vi "laser_power_measurement.vi"(1 "stop":bool) -> (0 "Readings":T1(array[cluster]) {"value" format="%#_6p"; "timestamp" format="%#.3f"})   [LabVIEW 2025]
panel:
  out "Device S/Ns":string[](array[string])
  out "Selected device S/N":string
  in  "OphirLMMeasurementLib.ICoLMMeasurement2":refnum<k7>
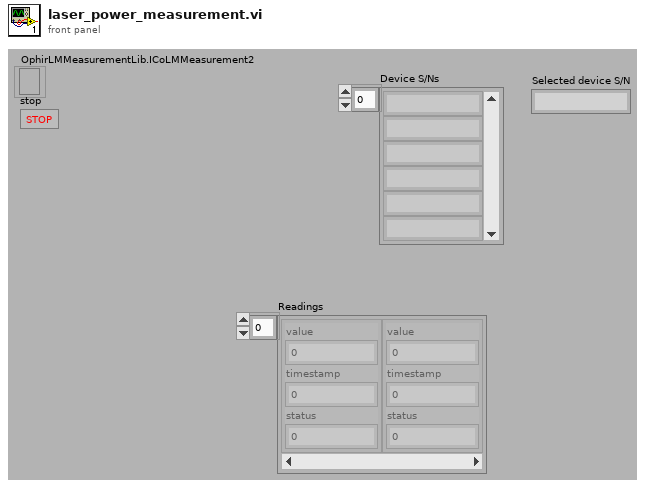
[diagram p1: front panel]
types:
  T1 = cluster{"value":dbl, "timestamp":dbl, "status":i32}[]
  T2 = cluster{"value":dbl, "timestamp":dbl, "status":i32}
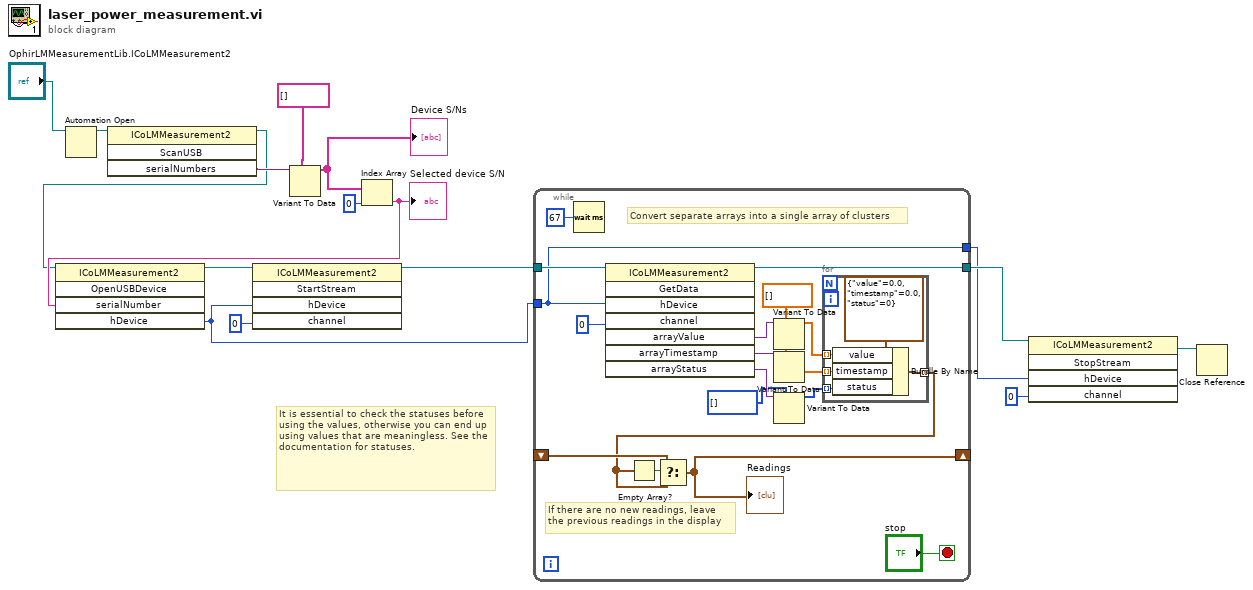
[diagram p0: block diagram]
diagram:
  # "It is essential to check the statuses before using the values, otherwise you can end up using values that are meaningless. See the documentation for statuses."
  n1 = Automation Open(Automation Refnum="OphirLMMeasurementLib.ICoLMMeasurement2") -> (Automation Refnum=w15:refnum<k7>)  [unwired: 3 in, 1 out]
  n2 = invoke class="ICoLMMeasurement2" method="ScanUSB"(reference=w15) -> (reference out=w9:refnum<k7>, "serialNumbers"=w14:variant)  [unwired: 3 in, 2 out]
  n3 = Variant To Data(type=string[] [], Variant=w14) -> (data=w13:string[])  [unwired: 1 in, 1 out]
  "Device S/Ns" <- w13
  n4 = Index Array(array=w13, index=0) -> (element=w10:string)
  "Selected device S/N" <- w10
  n5 = invoke class="ICoLMMeasurement2" method="OpenUSBDevice"(reference=w9, "serialNumber"=w10) -> (reference out=w8:refnum<k7>, "hDevice"=w6:i32)  [unwired: 3 in, 3 out]
  n6 = invoke class="ICoLMMeasurement2" method="StartStream"(reference=w8, "hDevice"=w6, "channel"=0) -> (reference out=w7:refnum<k7>)  [unwired: 2 in, 4 out]
  n7 = while {
    tunnel: w7 -> [w33]
    tunnel: w6 -> [w29]
    tunnel: [w30] -> w4
    tunnel: [w29] -> w3
    shift-right: [w20] -> _
    shift-left: _ -> [w19]
    stop <- "stop" stop-if-true
    w28 = dbl[] []
    # "Convert separate arrays into a single array of clusters"
    # "If there are no new readings, leave\nthe previous readings in the display"
    n8 = Wait (ms)(milliseconds to wait=u32 67) -> ()  [unwired: 1 out]
    n9 = invoke class="ICoLMMeasurement2" method="GetData"(reference=w33, "hDevice"=w29, "channel"=0) -> (reference out=w30:refnum<k7>, "arrayValue"=w27:variant, "arrayTimestamp"=w26:variant, "arrayStatus"=w25:variant)  [unwired: 5 in, 4 out]
    n10 = Variant To Data(type=w28, Variant=w27) -> (data=w24:dbl[])  [unwired: 1 in, 1 out]
    n11 = Variant To Data(type=w28, Variant=w26) -> (data=w23:dbl[])  [unwired: 1 in, 1 out]
    n12 = Variant To Data(type=i32[] [], Variant=w25) -> (data=w22:i32[])  [unwired: 1 in, 1 out]
    n13 = for {
      tunnel: w24 -> [w38] mode=indexing
      tunnel: w23 -> [w37] mode=indexing
      tunnel: w22 -> [w36] mode=indexing
      tunnel: [w35] -> w17 mode=indexing
      n14 = Bundle By Name(cluster=T2 {"value"=0.0, "timestamp"=0.0, "status"=0}, "value"=w38, "timestamp"=w37, "status"=w36) -> (w35:T2)
    }
    n15 = Empty Array?(array=w17) -> (empty?=w18:bool)
    n16 = Select(t=w19, s=w18, f=w17) -> (s? t:f=w20:T1)
    "Readings" <- w20
  }
  n17 = invoke class="ICoLMMeasurement2" method="StopStream"(reference=w4, "hDevice"=w3, "channel"=0) -> (reference out=w1:refnum<k7>)  [unwired: 2 in, 4 out]
  n18 = Close Reference(reference=w1) -> ()  [unwired: 1 in, 1 out]
